vi "Resolve New State.vi"(8 "error in":errorcluster, 9 "Assert Event Data":T1={"name"="", "passed"=FALSE, "call-chain"=[], "test-error"={"status"=FALSE, "code"=0, "source"=""}, "timestamp"=timestamp(0 s since 1904-01-01), "assert-id"="", "test-id"="", "time"=-1.0, "message"="", "properties"=variant, "measurements"=variant, "user-defined"=variant}, 11 "Current State":T2) -> (0 "error out":errorcluster, 3 "New State":T2)   [LabVIEW 2020, in "Caraya.lvlib" / "Basic Test Manager.lvclass"]
uses:
  Basic Test Manager.lvclass
  Test State.ctl
  Test Result/Assert Event Data (Extended).ctl
  Test Result/Test Result.lvclass
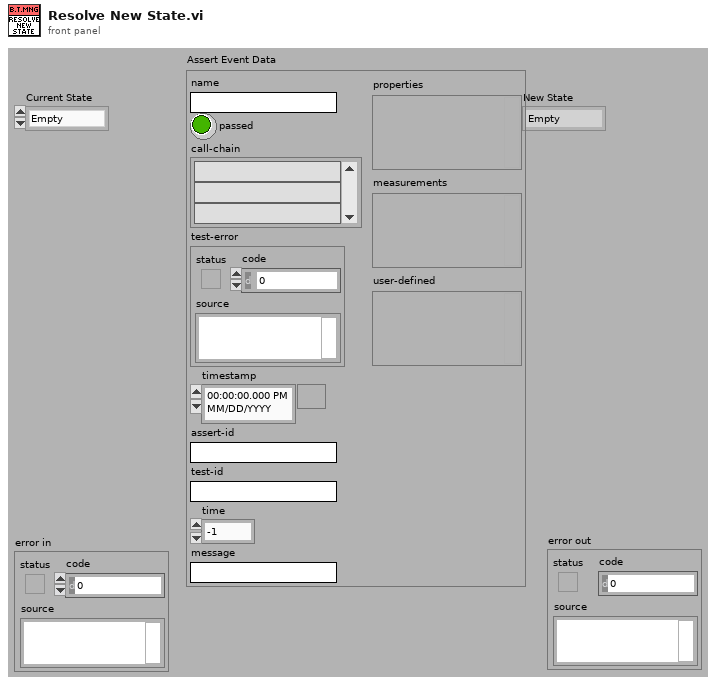
[diagram p1: front panel]
types:
  T1 = typedef "Caraya.lvlib/Test Result.lvclass/Assert Event Data (Extended).ctl" = cluster{"name":string, "passed":bool, "call-chain":string[], "test-error":errorcluster, "timestamp":timestamp, "assert-id":string, "test-id":string, "time":dbl, "message":string, "properties":variant, "measurements":variant, "user-defined":variant}
  T2 = typedef "Caraya.lvlib/Basic Test Manager.lvclass/Test State.ctl" = enum16{"Empty", "Unknown", "Fail", "Pass", "Skip", "Error"}
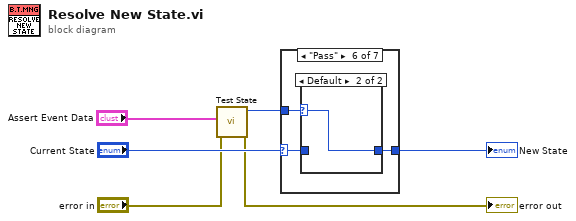
[diagram p0: block diagram]
diagram:
  n1 = call "Test State.vi"("error in (no error)"="error in", "Assert Event Data"="Assert Event Data") -> ("error out"=→"error out":errorcluster, "Test State"=w5:T2)  [unwired: 8 in]
  n2 = case shown="\"Pass\"" "Current State" {
    selector: "Current State" -> [w7 _ w9 _ w12 w17 _]
    tunnel: w5 -> [_ w8 _ w10 w13 w18 w21]
    tunnel: [w7 w8 w9 w10 w11 w16 w21] -> w6
    frame "Empty" {
    }
    frame "Unknown" {
    }
    frame "Fail" {
    }
    frame "Skip" {
    }
    frame "Error" {
      n3 = case shown="\"Fail\"" w13 {
        selector: w13 -> [_ w15]
        tunnel: w12 -> [w14 _]
        tunnel: [w14 w15] -> w11
        frame Default {
        }
        frame "Fail" {
        }
      }
    }
    frame "Pass" {
      n4 = case shown="Default" w18 {
        selector: w18 -> [_ w20]
        tunnel: w17 -> [w19 _]
        tunnel: [w19 w20] -> w16
        frame "Skip" {
        }
        frame Default {
        }
      }
    }
    frame Default {
    }
  }
  "New State" <- w6
